vi "Read Time Entry File.vi"(8 "error in (no error)":errorcluster, 11 "File Path":path) -> (0 "error out":errorcluster, 1 "Task Names":string[](array[string]), 2 "Project Names":string[](array[string]), 3 "Time Entries":T1)   [LabVIEW 2026]
doc: "Reads one month file (YYYY-MM.ini) and returns its time entries sorted by Start Time, with the Project Name and Task Name labels of each entry in the same order. An empty End Time becomes timestamp 0 (a running entry). The labels are returned only so that Write Time Entry File.vi can keep them - nothing should rely on them; IDs are the authority. A file that does not exist returns empty arrays and no error; a malformed timestamp returns error 5001.\n\nGenerated by: Claude"
uses:
  Rows/Time Entry List.ctl
  Rows/Time Entry.ctl
  Utilities/Time Management/Time Management.lvlib
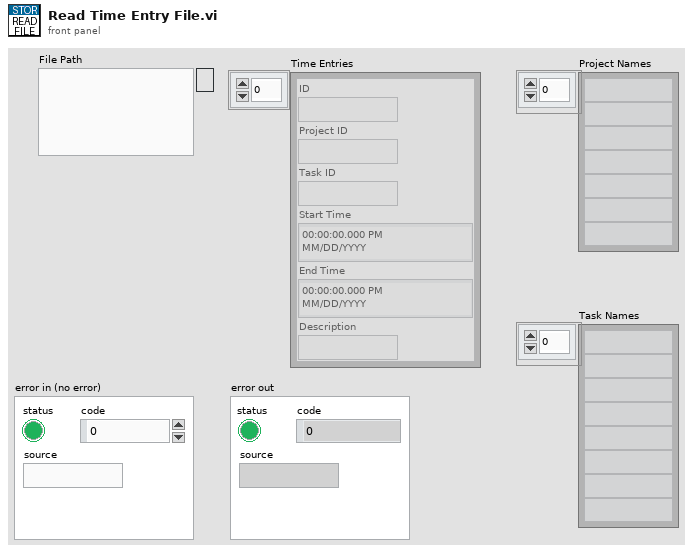
[diagram p1: front panel]
types:
  T1 = typedef "Time Entry List.ctl" = T2[]
  T2 = typedef "Time Entry.ctl" = cluster{"ID":string, "Project ID":string, "Task ID":string, "Start Time":timestamp, "End Time":timestamp, "Description":string}
  T3 = cluster{"String":string, string, string, "Timestamp":timestamp, "Timestamp":timestamp, string}
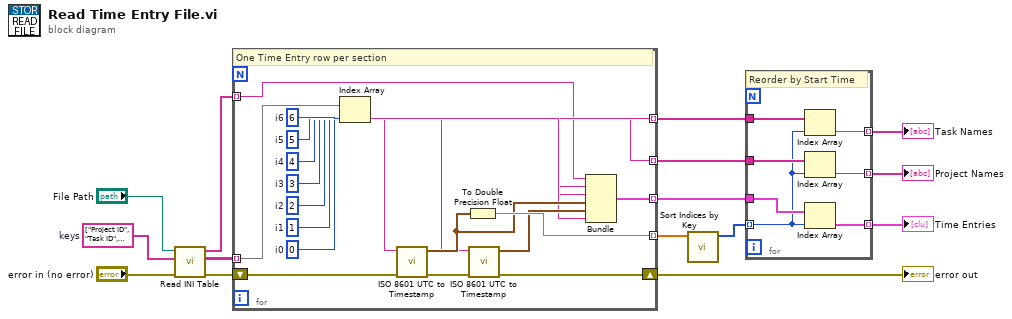
[diagram p0: block diagram]
diagram:
  w3 = string[] ["Project ID", "Task ID", "Project Name", "Task Name", "Start Time", "End Time", "Description"]  # keys
  n1 = call "Read INI Table.vi"("error in (no error)"="error in (no error)", "Keys"=w3, "File Path"="File Path") -> ("error out"=w6:errorcluster, "Values"=w5:string[][], "Section Names"=w4:string[])  [unwired: 6 in]
  n2 = for {
    tunnel: w4 -> [w16] mode=indexing
    tunnel: w5 -> [w17] mode=indexing
    shift-right: [w19] -> w7
    shift-left: w6 -> [w18]
    tunnel: [w29] -> w9 mode=indexing
    tunnel: [w30] -> w10 mode=indexing
    tunnel: [w38] -> w11 mode=indexing
    tunnel: [w37] -> w8 mode=indexing
    w26 = 6  # i6
    w25 = 5  # i5
    w24 = 4  # i4
    w23 = 3  # i3
    w22 = 2  # i2
    w21 = 1  # i1
    w20 = 0  # i0
    # "One Time Entry row per section"
    n3 = Index Array(array=w17, index #1=w20, index #2=w21, index #3=w22, index #4=w23, index #5=w24, index #6=w25, index #7=w26) -> (element #1=w27:string, element #2=w28:string, element #3=w29:string, element #4=w30:string, element #5=w31:string, element #6=w32:string, element #7=w33:string)
    n4 = call "ISO 8601 UTC to Timestamp.vi"("error in (no error)"=w18, "ISO 8601 UTC"=w31) -> ("error out"=w35:errorcluster, "Timestamp"=w34:timestamp)  [unwired: 8 in]
    n5 = To Double Precision Float(number=w34) -> (double precision float=w38:dbl)
    n6 = call "ISO 8601 UTC to Timestamp.vi"("error in (no error)"=w35, "ISO 8601 UTC"=w32) -> ("error out"=w19:errorcluster, "Timestamp"=w36:timestamp)  [unwired: 8 in]
    n7 = Bundle("String"=w16, w27, w28, "Timestamp"=w34, "Timestamp"=w36, w33) -> (w37:T3)  [unwired: 1 in]
  }
  "error out" <- w7
  n8 = call "Sort Indices by Key.vi"("Keys"=w11) -> ("Sorted Indices"=w12:i32[])  [unwired: 9 in, 1 out]
  n9 = for {
    tunnel: w9 -> [w41]
    tunnel: w10 -> [w42]
    tunnel: w12 -> [w39] mode=indexing
    tunnel: w8 -> [w40]
    tunnel: [w43] -> w13 mode=indexing
    tunnel: [w44] -> w14 mode=indexing
    tunnel: [w45] -> w15 mode=indexing
    # "Reorder by Start Time"
    n10 = Index Array(array=w42, index=w39) -> (element=w45:string)
    n11 = Index Array(array=w41, index=w39) -> (element=w44:string)
    n12 = Index Array(array=w40, index=w39) -> (element=w43:T3)
  }
  "Time Entries" <- w13
  "Project Names" <- w14
  "Task Names" <- w15
